vi "Table_Sort.vi"(7 "Sort Type":enum16{"numerical", "hex", "string"}(ring), 9 "Sort by":u16(ring) items=["Packet_Number", "Timestamp", "Source", "Destination", "Protocol", "Length", "Data"], 11 "Unsorted Data":string[][](array[string])=array1500x7[10500 elements]) -> (3 "Sorted data":string[][](array[string]))   [LabVIEW 2025, in "Table_Filtering.lvlib"]
uses:
  Table_Filtering.lvlib
  dd903b07-9a56-4d29-89d8-b4a603456dcb.vi
  <vilib>/Array/Sort 2D Array - Pop Stack.vi
  <vilib>/Array/Sort 2D Array - Push Stack.vi
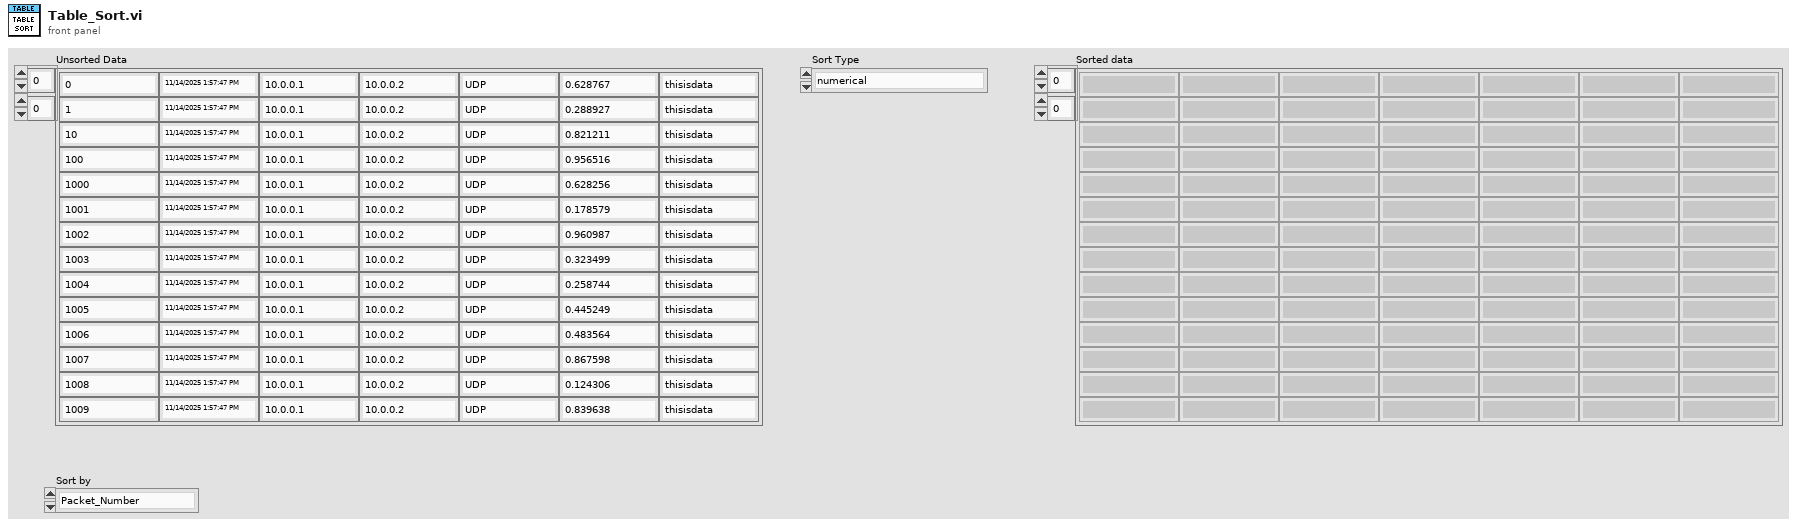
[diagram p1: front panel]
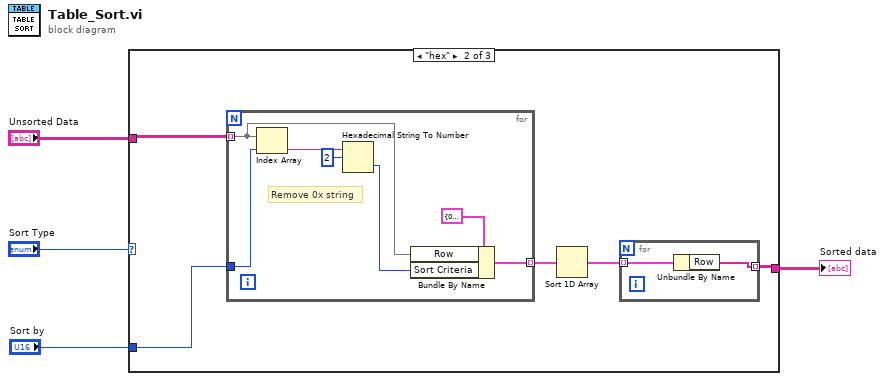
[diagram p0: block diagram]
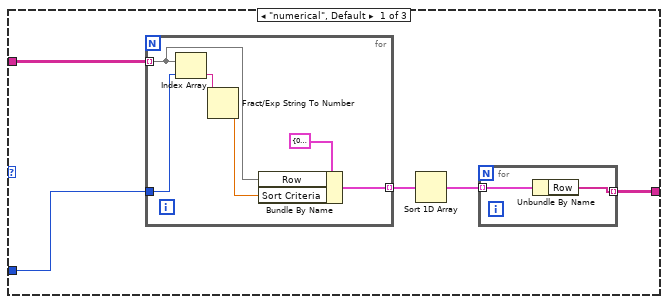
[diagram p2: hidden frame]
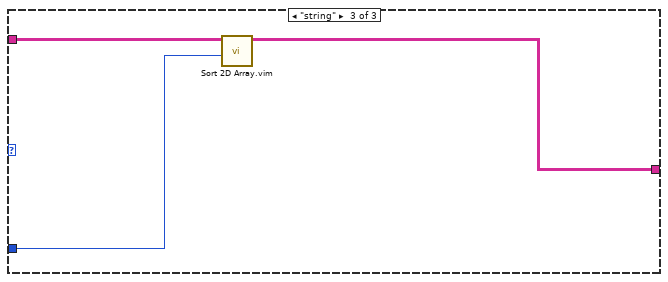
[diagram p3: hidden frame]
diagram:
  n1 = case shown="\"hex\"" "Sort Type" {
    tunnel: "Unsorted Data" -> [w9 w18 w34]
    tunnel: "Sort by" -> [w8 w19 w32]
    tunnel: [w5 w20 w33] -> w1
    frame "numerical", Default {
      n2 = for {
        tunnel: w9 -> [w12] mode=indexing
        tunnel: w8 -> [w13]
        tunnel: [w10] -> w7 mode=indexing
        n3 = Index Array(array=w12, index=w13) -> (element=w15:string)
        n4 = Fract/Exp String To Number(string=w15) -> (number=w11:dbl)  [unwired: 3 in, 1 out]
        n5 = Bundle By Name(cluster=cluster{"Sort Criteria":dbl, "Row":string[]} {"Sort Criteria"=0.0, "Row"=[]}, "Row"=w12, "Sort Criteria"=w11) -> (w10:cluster{"Sort Criteria":dbl, "Row":string[]})
      }
      n6 = Sort 1D Array(array=w7) -> (sorted array=w6:cluster{"Sort Criteria":dbl, "Row":string[]}[])
      n7 = for {
        tunnel: w6 -> [w17] mode=indexing
        tunnel: [w16] -> w5 mode=indexing
        n8 = Unbundle By Name(w17) -> ("Row"=w16:string[])
      }
    }
    frame "hex" {
      n9 = for {
        tunnel: w18 -> [w27] mode=indexing
        tunnel: w19 -> [w28]
        tunnel: [w26] -> w22 mode=indexing
        # "Remove 0x string"
        n10 = Index Array(array=w27, index=w28) -> (element=w24:string)
        n11 = Hexadecimal String To Number(string=w24, offset=2) -> (number=w25:u32)  [unwired: 1 in, 1 out]
        n12 = Bundle By Name(cluster=cluster{"Sort Criteria":dbl, "Row":string[]} {"Sort Criteria"=0.0, "Row"=[]}, "Row"=w27, "Sort Criteria"=w25) -> (w26:cluster{"Sort Criteria":dbl, "Row":string[]})
      }
      n13 = Sort 1D Array(array=w22) -> (sorted array=w21:cluster{"Sort Criteria":dbl, "Row":string[]}[])
      n14 = for {
        tunnel: w21 -> [w31] mode=indexing
        tunnel: [w30] -> w20 mode=indexing
        n15 = Unbundle By Name(w31) -> ("Row"=w30:string[])
      }
    }
    frame "string" {
      n16 = call "Sort 2D Array.vim"("index"=w32, "2D array"=w34) -> ("sorted 2D array"=w33:string[][])  [unwired: 8 in, 1 out]
    }
  }
  "Sorted data" <- w1
